vi "Test Add Clears Redo.vi"(8 "error in":errorcluster, 11 "Test Case In":refnum<class "History Tests.lvclass">) -> (0 "error out":errorcluster, 3 "Test Case Out":refnum<class "History Tests.lvclass">)   [LabVIEW 2020, in "History Tests.lvclass"]
uses:
  History Tests.lvclass
  History Tests.lvclass/History Tests.ctl
  C:/Program Files/National Instruments/LabVIEW 2026/vi.lib/Astemes/LUnit/Test Case.lvclass
  C:/Program Files/National Instruments/LabVIEW 2026/vi.lib/Astemes/LUnit/LUnit Runnable.lvclass
  C:/Users/J63553/Projects/_LabVIEW Community/labview-icon-editor/Test/Unit Tests/History Tests/History Tests.lvclass
  d374c4ae-0456-4ebf-b145-8753cc394ed2.vi
  <vilib>/Astemes/LUnit/Test Case.lvclass
  resource/plugins/NIIconEditor/History/History/History.lvclass
  5d03536d-b951-4893-9e85-05bb1b57c72f.vi
panel:
  out "State After Redo":string
  out "State After Adding":string
  out "Undo State Outputs":string[](array[string])
  out "State After Initial Adding":string
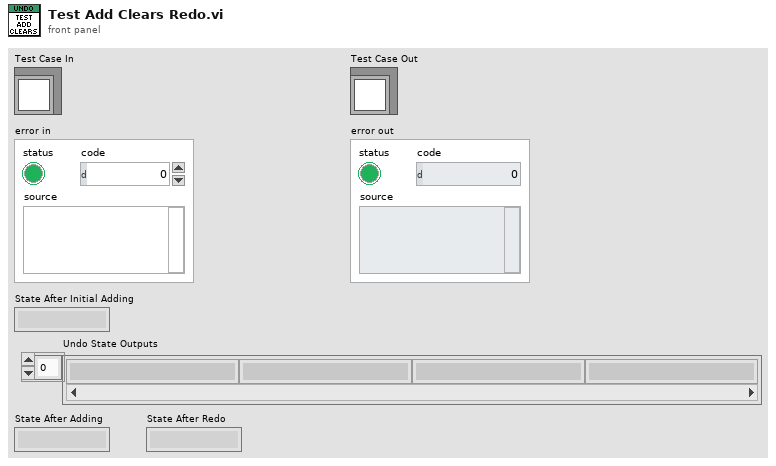
[diagram p1: front panel]
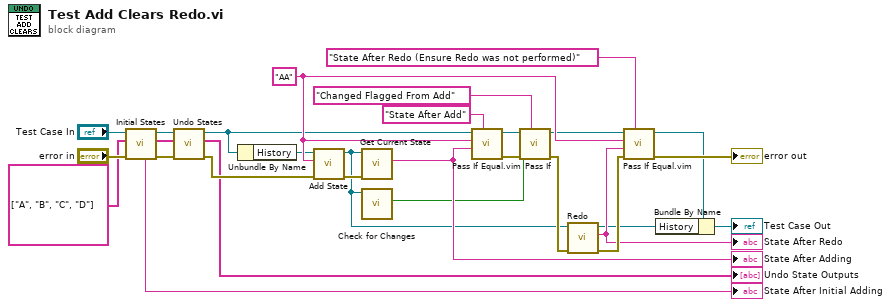
[diagram p0: block diagram]
diagram:
  w21 = "AA" ("Data in")
  n1 = call "Initial States.vi"("error in"="error in", "States"=string[] ["A", "B", "C", "D"], "Test Case In"="Test Case In") -> ("error out"=w29:errorcluster, "Expected Undo Stack"=w14:string[], "Test Case Out"=w17:refnum<class "History Tests.lvclass">, "Current State"=→"State After Initial Adding":string)  [unwired: 5 in]
  n2 = call "Undo States.vi"("error in"=w29, "Expected Undo States"=w14, "Test Case In"=w17) -> ("error out"=w27:errorcluster, "Actual Undo States"=→"Undo State Outputs":string[], "Test Case Out"=w9:refnum<class "History Tests.lvclass">)  [unwired: 6 in]
  n3 = Unbundle By Name(w9) -> ("History"=w8:refnum<class "History.lvclass">)
  n4 = call "Add State.vi"("error in"=w27, "State"=w21, "History in"=w8) -> ("error out"=w26:errorcluster, "History out"=w4:refnum<class "History.lvclass">)  [unwired: 7 in]
  n5 = call "Get Current State.vi"("error in"=w26, "History"=w4) -> ("Current State"=w7:string)  [unwired: 7 in, 2 out]
  "State After Adding" <- w7
  n6 = call "Check for Changes.vi"("History"=w4) -> ("Have Changes"=w6:bool)  [unwired: 10 in]
  n7 = call "Pass If Equal.vim"("Description"="State After Add", "Actual"=w7, "Expected"=w21, "LUnit Test Case In"=w9) -> ("error out"=w28:errorcluster, "LUnit Test Case Out"=w12:refnum<class "History Tests.lvclass">)  [unwired: 6 in]
  n8 = call <vilib>:"Pass If.vi"("Description"="Changed Flagged From Add", "error in (no error)"=w28, "Pass?"=w6, "LUnit Test Case In"=w12) -> ("error out"=w25:errorcluster, "LUnit Test Case Out"=w11:refnum<class "History Tests.lvclass">)  [unwired: 6 in]
  n9 = call "Redo.vi"("error in"=w25, "History in"=w4) -> ("error out"=w24:errorcluster, "State"=w5:string, "History out"=w2:refnum<class "History.lvclass">)  [unwired: 7 in]
  "State After Redo" <- w5
  n10 = call "Pass If Equal.vim"("Description"="State After Redo (Ensure Redo was not performed)", "error in (no error)"=w24, "Actual"=w5, "Expected"=w21, "LUnit Test Case In"=w11) -> ("error out"=→"error out":errorcluster, "LUnit Test Case Out"=w3:refnum<class "History Tests.lvclass">)  [unwired: 5 in]
  n11 = Bundle By Name(cluster=w3, "History"=w2) -> (→"Test Case Out":refnum<class "History Tests.lvclass">)
